vi "List Local Chassis Modules.vi"(8 "error in (no error)":errorcluster, 11 "Item Ref in":T1 format="%.0x") -> (0 "error out":errorcluster, 2 "Local Slots #":u32[](array[numeric]), 3 "Item Ref out":T1 format="%.0x")   [LabVIEW 2017, in "Scan Engine Custom Device.lvlib"]
doc: "This VI lists the module(s) configured in Local Chassis. GUIDs are used to create the list. The output is a list of Slot Number."
uses:
  Scan Engine Custom Device.lvlib
  <vilib>/NI Veristand/Custom Device API/Custom Device Item Ref.ctl
  Globals/Scan Engine GUIDs.vi
  <vilib>/NI Veristand/Custom Device Tools/Custom Device Utility Library/NI VeriStand - Search for Item by GUID.vi
  <vilib>/NI Veristand/Custom Device Tools/Custom Device Utility Library/NI VeriStand - Search for All Items by GUID.vi
  <vilib>/NI Veristand/Custom Device Tools/Custom Device Utility Library/Custom Device Utility Library.lvlib
  Modules.lvlibp/RSI Module/RSI Module.lvclass
  <vilib>/NI Veristand/Custom Device API/Custom Device API.lvlib
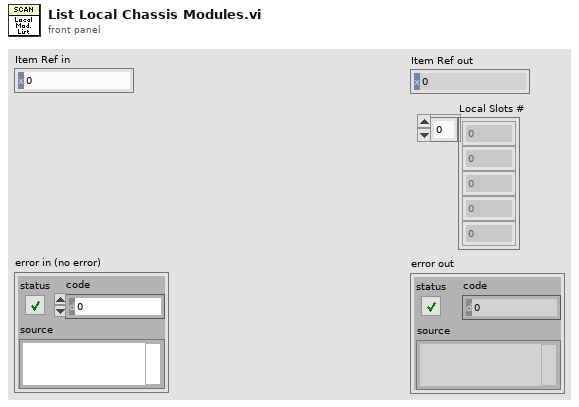
[diagram p1: front panel]
types:
  T1 = typedef "Custom Device API.lvlib/Custom Device Item Ref.ctl" = u64
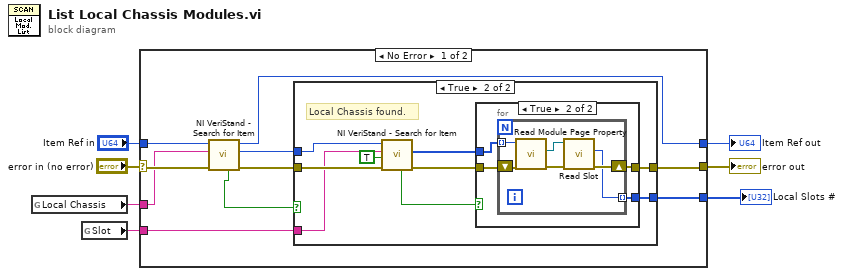
[diagram p0: block diagram]
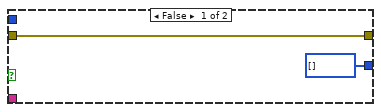
[diagram p2: hidden frame]
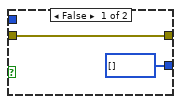
[diagram p3: hidden frame]
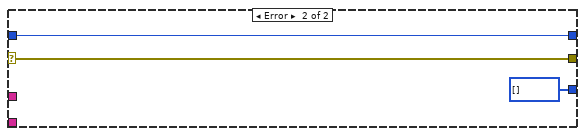
[diagram p4: hidden frame]
diagram:
  n1 = global read "Scan Engine GUIDs.vi" "Local Chassis"() -> (w4:string)
  n2 = global read "Scan Engine GUIDs.vi" "Slot"() -> (w2:string)
  n3 = case shown="No Error" "error in (no error)" {
    selector: "error in (no error)" -> [w17 w43]
    tunnel: [w9 w43] -> w6
    tunnel: "Item Ref in" -> [w16 w42]
    tunnel: w4 -> [w15 _]
    tunnel: [w11 w42] -> w3
    tunnel: w2 -> [w10 _]
    tunnel: [w8 u32[] []] -> w1
    frame No Error {
      n4 = call-poly <vilib>:"NI VeriStand - Search for Item.vi"("error in"=w17, "Item GUID"=w15, "Section Ref in"=w16) -> ("error out"=w13:errorcluster, "Item Ref"=w12:T1, "Section Ref out"=w11:T1, "Found"=w14:bool)  [unwired: 5 in]
      n5 = case shown="True" w14 {
        tunnel: w13 -> [w18 w28]
        tunnel: w12 -> [_ w27]
        tunnel: w10 -> [_ w26]
        tunnel: [w18 w22] -> w9
        tunnel: [u32[] [] w20] -> w8
        frame False {
        }
        frame True {
          # "Local Chassis found."
          n6 = call-poly <vilib>:"NI VeriStand - Search for Item.vi"("error in"=w28, "Find All? (T)"=TRUE, "Item GUID"=w26, "Section Ref in"=w27) -> ("error out"=w23:errorcluster, "Item Refs"=w21:T1[], "Found"=w24:bool)  [unwired: 4 in, 1 out]
          n7 = case shown="True" w24 {
            tunnel: w23 -> [w30 w34]
            tunnel: [w30 w32] -> w22
            tunnel: w21 -> [_ w33]
            tunnel: [u32[] [] w31] -> w20
            frame False {
            }
            frame True {
              n8 = for {
                tunnel: w33 -> [w37] mode=indexing
                shift-right: [w36] -> w32
                shift-left: w34 -> [w40]
                tunnel: [w35] -> w31 mode=indexing
                n9 = call "Read Module Page Property.vi"("error in (no error)"=w40, "Node Ptr In"=w37) -> ("error out"=w39:errorcluster, "RSI Module"=w38:refnum<class "RSI Module.lvclass">)  [unwired: 7 in, 1 out]
                n10 = call "Read Slot.vi"("error in (no error)"=w39, "RSI Module in"=w38) -> ("error out"=w36:errorcluster, "Slot"=w35:u32)  [unwired: 7 in, 1 out]
              }
            }
          }
        }
      }
    }
    frame Error {
    }
  }
  "Item Ref out" <- w3
  "error out" <- w6
  "Local Slots #" <- w1
